vi "Apply Speed.vi"(8 "error in (no error)":errorcluster, 11 "Tool Rectangle in":refnum<class "Tool Rectangle.lvclass">) -> (0 "error out":errorcluster, 3 "Tool Rectangle out":refnum<class "Tool Rectangle.lvclass">)   [LabVIEW 2019, in "Tool Rectangle.lvclass"]
uses:
  Tool Rectangle.lvclass
  Settings/ObjectSettings/ObjectSettings.lvclass/ObjectSettings.ctl
  Settings/Rectangle Settings/Rectangle Settings.lvclass
  C:/Users/Albro/Documents/GitHub/AFM-Lithography/lvsrc/Classes/Settings/ObjectSettings/ObjectSettings.lvclass
  Settings/ObjectSettings/ObjectSettings.lvclass
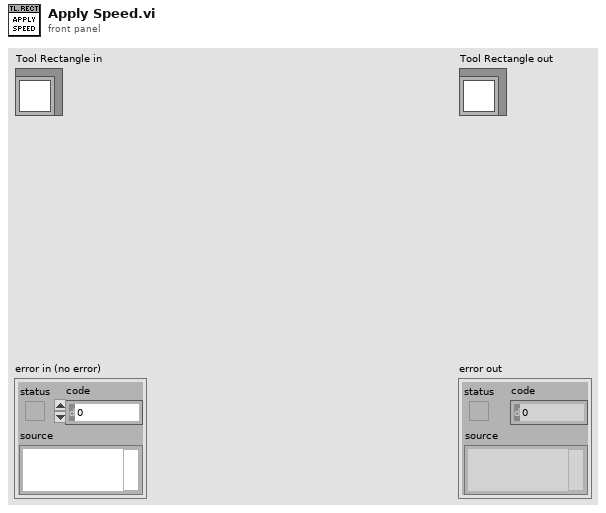
[diagram p1: front panel]
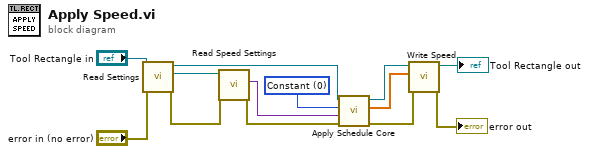
[diagram p0: block diagram]
diagram:
  w6 = u16 0 items=["Constant", "Ramp", "Function", "Formula"] ("Schedule")
  n1 = call-dynamic "Read Settings.vi"("error in (no error)"="error in (no error)", "Tool Rectangle in"="Tool Rectangle in") -> ("error out"=w8:errorcluster, "Rectangle Settings.lvclass"=w10:refnum<class "Rectangle Settings.lvclass">, "Tool Rectangle out"=w13:refnum<class "Tool Rectangle.lvclass">)  [unwired: 7 in]
  n2 = call "Read Speed Settings.vi"("error in (no error)"=w8, "ObjectSettings in"=w10) -> ("error out"=w7:errorcluster, "Settings"=w9:variant)  [unwired: 7 in, 1 out]
  n3 = call-dynamic "Apply Schedule Core.vi"("error in (no error)"=w7, "Settings"=w9, "Schedule"=w6, "Tool Object in"=w13) -> ("error out"=w2:errorcluster, "Schedule Array"=w3:dbl[], "Tool Object out"=w5:refnum<class "Tool Rectangle.lvclass">)  [unwired: 5 in]
  n4 = call-dynamic "Write Speed.vi"("error in (no error)"=w2, "Speed"=w3, "Tool Object in"=w5) -> ("error out"=→"error out":errorcluster, "Tool Object out"=→"Tool Rectangle out":refnum<class "Tool Rectangle.lvclass">)  [unwired: 7 in]
